vi "Measure Sound from Digital Mic - PDM and I2S.vi"() -> ()   [LabVIEW 2022 SP3]
doc: "This example performs a continuous acquisition of PCM data. At the same time, the GPIO lines are used for digital input and digital output."
uses:
  <vilib>/PDM Acquisition Toolkit/host/Classes/Tasks/PDM Tasks/Controls/Acquisition Mode.ctl
  <vilib>/PDM Acquisition Toolkit/shared/controls/clock mode.ctl
  <vilib>/addons/_NISVFA/_Shared subVIs/Common/SVL Set dB Reference (1 Ch).vi
  <vilib>/addons/Sound and Vibration/svt_Level/SVL AC & DC Level (Time) (1 Ch).vi
  <vilib>/addons/_NISVFA/_Shared subVIs/Common/SVL Set dB Reference (variant).vi
  <vilib>/addons/_NISVFA/_Shared subVIs/Common/svc_Get SV Channel Info.vi
  <vilib>/Analysis/baseanly.llb/Mean.vi
  <vilib>/Analysis/baseanly.llb/Mean (DBL).vi
  <vilib>/addons/_NISVFA/_Shared subVIs/Windowing/svfa_Scaled Time Domain Window (Array).vi
  <vilib>/addons/_NISVFA/_Shared subVIs/Common/svc_Unit Label to Engineering Units.vi
  <vilib>/addons/_NISVFA/_Shared subVIs/Common/svc_Engineering Units to Unit Label.vi
  <vilib>/addons/_NISVFA/_Spectrum Processing/subVIs/svfa_Spectrum Info Window to windowTd Type Def.vi
  <vilib>/Analysis/4window.llb/Force Window.vi
  <vilib>/Analysis/4window.llb/Force Window (DBL).vi
  <vilib>/Analysis/4window.llb/Exponential Window.vi
  <vilib>/Analysis/4window.llb/Exponential Window (DBL).vi
  <vilib>/addons/_NISVFA/_Shared subVIs/Common/svc_Caller VI Returned in Error Source.vi
  <vilib>/addons/_NISVFA/_Shared subVIs/Common/svc_Get Window Info.vi
  <vilib>/Analysis/0measdsp.llb/Scaled Time Domain Window.vi
  <vilib>/Analysis/0measdsp.llb/Scaled Time Domain Window (DBL).vi
  <vilib>/Utility/error.llb/Error Cluster From Error Code.vi
  <vilib>/Analysis/baseanly.llb/Std Deviation and Variance.vi
  <vilib>/addons/Sound and Vibration/svt_Weighting/SVT Weighting Filter (1 Ch).vi
  <vilib>/addons/Sound and Vibration/svt_Level/SVL Leq Sound Level (1 Ch).vi
  <vilib>/PDM Acquisition Toolkit/host/Classes/Tasks/PDM Tasks/PDM Task.lvclass
  <vilib>/PDM Acquisition Toolkit/shared/PDM Shared.lvlib
  <vilib>/addons/Sound and Vibration/svt_Weighting/SoundVib_ABCWeighting.lvlib
  <vilib>/addons/Sound and Vibration/svt_Level/SoundVib_SoundLevel.lvlib
  source/shared/combined digital api/Combo Digital Audio API.lvlib
panel:
  in  "File Path":path=path "C:/dev/digital-microphone/test/test-I2S.inputcfg"
  out "Leq sound level [dB EU]":dbl=94.84187633004404 format="%.2f"
  in  "weighting":u16(ring) items=["Linear", "A-weighting", "B-weighting", "C-weighting"]
  out "Error Out":errorcluster
  out "Waveform Graph":waveform(dbl)(graph)={"t0"=timestamp(0 s since 1904-01-01), "dt"=2.0833333110203966e-05, "Y"=[], "attributes"=variant("NI_ChannelName"=variant(string "PCMI8.0"), "NI_dBReference"=variant(dbl 2e-05))}
  in  "Acquisition duration (s)":dbl=12000.0
  in  "PDM Channels":string="PXI1Slot5\\PCMi 8"
  in  "Microphone Sensitivity (dBFS)":dbl=-26.0 format="%#_13g"
  in  "Stop":bool
  # "PDM Input"
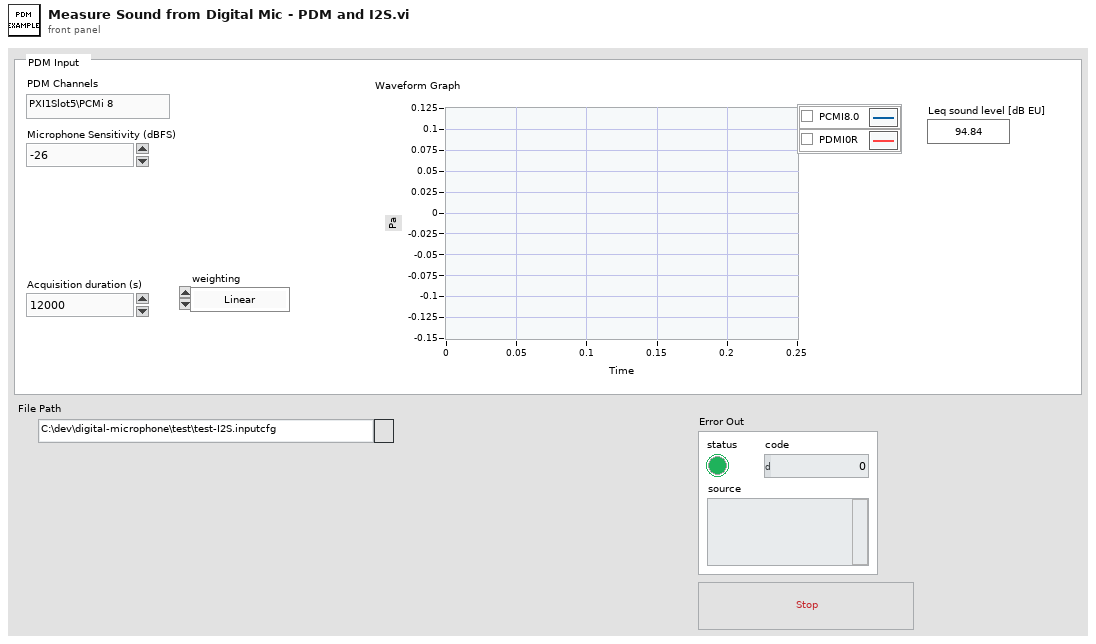
[diagram p1: front panel]
types:
  T1 = typedef "PDM Shared.lvlib/clock mode.ctl" = enum16{"divided clock", "DDS"}
  T2 = typedef "PDM Acquisition Class Library.lvlib/PDM Task.lvclass/Acquisition Mode.ctl" = enum16{"Finite", "Continuous"}
  T3 = typedef "Combo Digital Audio API.lvlib/task.ctl" = cluster{"task ref":u64, "audio type":T4, "sample rate":dbl}
  T4 = typedef "input type.ctl" = enum32{"Digital Serial", "PDM"}
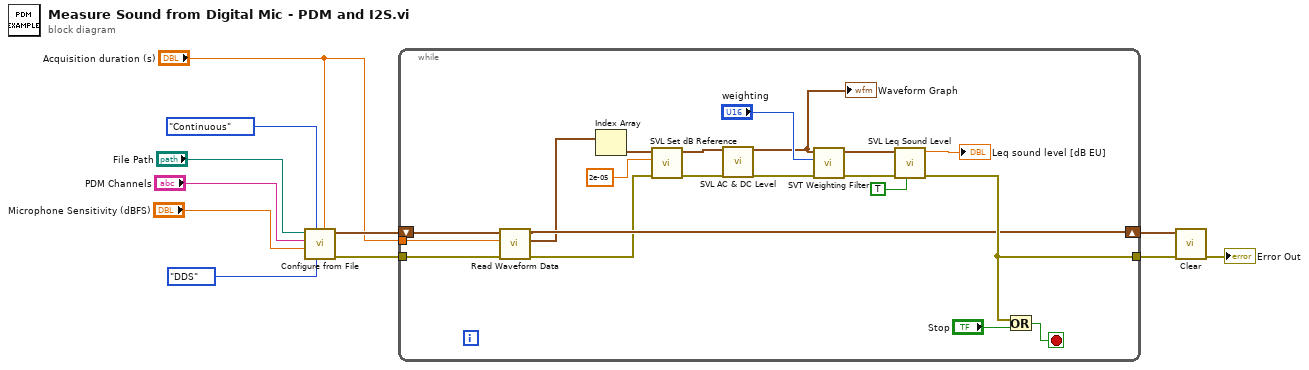
[diagram p0: block diagram]
diagram:
  n1 = call "Configure from File.vi"("acq duration (s)"="Acquisition duration (s)", "clock mode"=clock_mode."DDS", "acquisition mode"=Acquisition_Mode."Continuous", "microphone sensitivity (dBFS)"="Microphone Sensitivity (dBFS)", "channels"="PDM Channels", "file path"="File Path") -> ("error out"=w11:errorcluster, "task"=w10:T3)  [unwired: 4 in]
  n2 = while {
    tunnel: w11 -> [w17]
    tunnel: "Acquisition duration (s)" -> [w15]
    shift-right: [w14] -> w2
    shift-left: w10 -> [w16]
    tunnel: [w18] -> w3
    stop <- w31 stop-if-true
    n3 = call "Read Waveform Data.vi"("error in (no error)"=w17, "acq duration (s)"=w15, "task"=w16) -> ("error out"=w13:errorcluster, "waveforms"=w12:waveform(dbl)[], "task"=w14:T3)  [unwired: 6 in]
    n4 = Index Array(array=w12) -> (element=w24:waveform(dbl))  [unwired: 1 in]
    n5 = call-poly <vilib>:"SVL Set dB Reference.vi"("error in (no error)"=w13, "dB reference [EU]"=2e-05, "scaled signal in [EU]"=w24) -> ("error out"=w19:errorcluster, "scaled signal out [EU]"=w22:waveform(dbl))  [unwired: 7 in]
    n6 = call-poly <vilib>:"SVL AC & DC Level.vi"("scaled signal [EU]"=w22, "error in (no error)"=w19) -> ("AC signal [EU]"=w21:waveform(dbl), "error out"=w20:errorcluster)  [unwired: 12 in, 4 out]
    "Waveform Graph" <- w21
    n7 = call-poly <vilib>:"SVT Weighting Filter.vi"("error in (no error)"=w20, "weighting"="weighting", "scaled signal [EU]"=w21) -> ("error out"=w28:errorcluster, "weighted signal [EU]"=w25:waveform(dbl))  [unwired: 6 in]
    n8 = call-poly <vilib>:"SVL Leq Sound Level.vi"("restart averaging (F)"=TRUE, "error in (no error)"=w28, "scaled signal [EU]"=w25) -> ("error out"=w18:errorcluster, "Leq sound level [dB EU]"=→"Leq sound level [dB EU]":dbl)  [unwired: 6 in, 1 out]
    n9 = Or(x=w18, y="Stop") -> (x .or. y?=w31:bool)
  }
  n10 = call "Clear.vi"("error in (no error)"=w3, "task"=w2) -> ("error out"=→"Error Out":errorcluster)  [unwired: 9 in]
